vi "Sound conversion (16b, mono).vi"(4 "stereo 8-bit":u8[][](array[numeric]), 5 "mono 8-bit":u8[](array[numeric]), 6 "stereo 16-bit":i16[][](array[numeric]), 7 "mono 16-bit":i16[](array[numeric]), 8 "conver rate? (F)":bool, 9 "result rate":enum16{"11025", "22050", "44100"}(ring), 10 "wave format":T1) -> (1 "rate out":enum16{"11025", "22050", "44100"}(ring), 3 "sound out":i16[](array[numeric]))   [LabVIEW 2021]
doc: "::: CalcExpress Toolkit :::\nCopyright (c) 2000-2026 Konstantin Shifershteyn. All rights reserved."
uses:
  <vilib>/sound/lvsound.llb/Sound Format.ctl
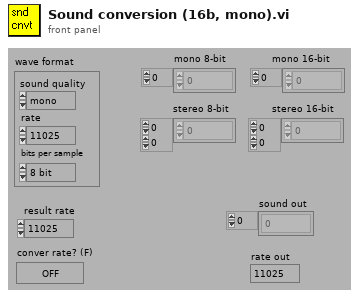
[diagram p1: front panel]
types:
  T1 = typedef "Sound Format.ctl" = cluster{"sound quality":enum16{"mono", "stereo"}, "rate":enum16{"11025", "22050", "44100", "8000"}, "bits per sample":enum16{"8 bit", "16 bit"}}
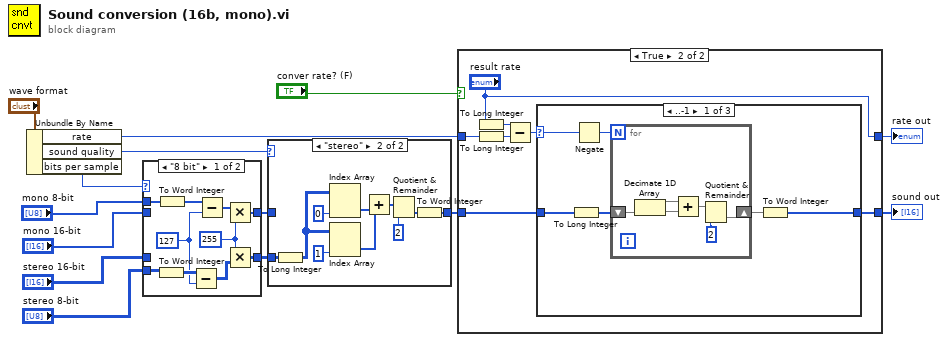
[diagram p0: block diagram]
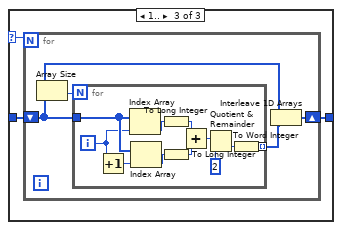
[diagram p4: hidden frame]
diagram:
  n1 = Unbundle By Name("wave format") -> ("rate"=w4:enum16{"11025", "22050", "44100", "8000"}, "sound quality"=w12:enum16{"mono", "stereo"}, "bits per sample"=w11:enum16{"8 bit", "16 bit"})
  n2 = case shown="\"8 bit\"" w11 {
    tunnel: "mono 16-bit" -> [_ w26]
    tunnel: "mono 8-bit" -> [w24 _]
    tunnel: "stereo 16-bit" -> [_ w25]
    tunnel: "stereo 8-bit" -> [w20 _]
    tunnel: [w19 w26] -> w13
    tunnel: [w17 w25] -> w14
    frame "8 bit" {
      w16 = i16 255
      w15 = i16 127
      n3 = To Word Integer(number=w20) -> (16bit integer=w21:i16[][])
      n4 = To Word Integer(number=w24) -> (16bit integer=w23:i16[])
      n5 = Subtract(x=w21, y=w15) -> (x-y=w22:i16[][])
      n6 = Subtract(x=w23, y=w15) -> (x-y=w18:i16[])
      n7 = Multiply(x=w18, y=w16) -> (x*y=w19:i16[])
      n8 = Multiply(x=w16, y=w22) -> (x*y=w17:i16[][])
    }
    frame "16 bit", Default {
    }
  }
  n9 = case shown="\"stereo\"" w12 {
    tunnel: w13 -> [w27 _]
    tunnel: [w27 w28] -> w5
    tunnel: w14 -> [_ w37]
    frame "mono", Default {
    }
    frame "stereo" {
      n10 = To Long Integer(number=w37) -> (32bit integer=w29:i32[][])
      n11 = Index Array(array=w29, index (col)=0) -> (element=w36:i32[])  [unwired: 1 in]
      n12 = Index Array(array=w29, index (col)=1) -> (element=w35:i32[])  [unwired: 1 in]
      n13 = Add(x=w36, y=w35) -> (x+y=w34:i32[])
      n14 = Quotient & Remainder(x=w34, y=2) -> (floor(x/y)=w32:i32[])  [unwired: 1 out]
      n15 = To Word Integer(number=w32) -> (16bit integer=w28:i16[])
    }
  }
  n16 = case shown="True" "conver rate? (F)" {
    tunnel: w5 -> [w39 w41]
    tunnel: w4 -> [w38 w44]
    tunnel: [w39 w40] -> w2
    tunnel: [w38 "result rate"] -> w1
    frame False {
    }
    frame True {
      n17 = To Long Integer(number="result rate") -> (32bit integer=w45:i32)
      n18 = To Long Integer(number=w44) -> (32bit integer=w46:i32)
      n19 = Subtract(x=w45, y=w46) -> (x-y=w42:i32)
      n20 = case shown="..-1" w42 {
        selector: w42 -> [w47 _ w61]
        tunnel: w41 -> [w52 w59 w62]
        tunnel: [w48 w59 w60] -> w40
        frame ..-1 {
          n21 = To Long Integer(number=w52) -> (32bit integer=w49:i32[])
          n22 = Negate(x=w47) -> (-x=w50:i32)
          n23 = for {
            N: w50 -> [_]
            shift-right: [w53] -> w51
            shift-left: w49 -> [w58]
            n24 = Decimate 1D Array(w58) -> (w57:i32[], w56:i32[])
            n25 = Add(x=w57, y=w56) -> (x+y=w55:i32[])
            n26 = Quotient & Remainder(x=w55, y=2) -> (floor(x/y)=w53:i32[])  [unwired: 1 out]
          }
          n27 = To Word Integer(number=w51) -> (16bit integer=w48:i16[])
        }
        frame 0 {
        }
        frame 1.. {
          n28 = for {
            N: w61 -> [_]
            shift-right: [w64] -> w60
            shift-left: w62 -> [w66]
            n29 = Array Size(array=w66) -> (size(s)=w63:i32)
            n30 = for {
              N: w63 -> [_]
              tunnel: w66 -> [w69]
              tunnel: [w68] -> w65 mode=indexing
              i -> [w67]
              n31 = Increment(x=w67) -> (x+1=w77:i32)
              n32 = Index Array(array=w69, index=w67) -> (element=w73:i16)
              n33 = Index Array(array=w69, index=w77) -> (element=w72:i16)
              n34 = To Long Integer(number=w73) -> (32bit integer=w70:i32)
              n35 = To Long Integer(number=w72) -> (32bit integer=w71:i32)
              n36 = Add(x=w70, y=w71) -> (x+y=w74:i32)
              n37 = Quotient & Remainder(x=w74, y=2) -> (floor(x/y)=w76:i32)  [unwired: 1 out]
              n38 = To Word Integer(number=w76) -> (16bit integer=w68:i16)
            }
            n39 = Interleave 1D Arrays(w66, w65) -> (w64:i16[])
          }
        }
      }
    }
  }
  "sound out" <- w2
  "rate out" <- w1
